vi "ZM-receiver.vi"() -> ()   [LabVIEW 2020]
doc: "UDP receiver of the tree's data: a plain top-level VI outside the actor tree, started and stopped at any time. It listens on port (default 61557), charts temperature_c and duty_percent of each test package, and shows the last line, the packet count and the measured interval; other package types are skipped. Stop or an error ends it and releases the port."
uses:
  protocol/ZM-CP-UDP-udp_transport/ZM-CP-UDP-receiver/ZM-CP-UDP-receiver.lvclass
  common/ZM-PC-packages/ZM-PC-package/ZM-PC-HEADER.ctl
  common/ZM-PC-packages/ZM-PC-package/ZM-PC-package.lvclass
  common/ZM-PC-packages/ZM-PC-TP-test_package/ZM-PC-TP-DATA.ctl
  common/ZM-PC-packages/ZM-PC-TP-test_package/ZM-PC-TP-test_package.lvclass
panel:
  out "error out":errorcluster
  in  "Stop":bool
  out "packets":u32
  out "last line":string
  out "interval measured (ms)":u32
  out "chart":cluster{"temperature_c":dbl, "duty_percent":dbl}(graph)
  in  "port":u16=61557
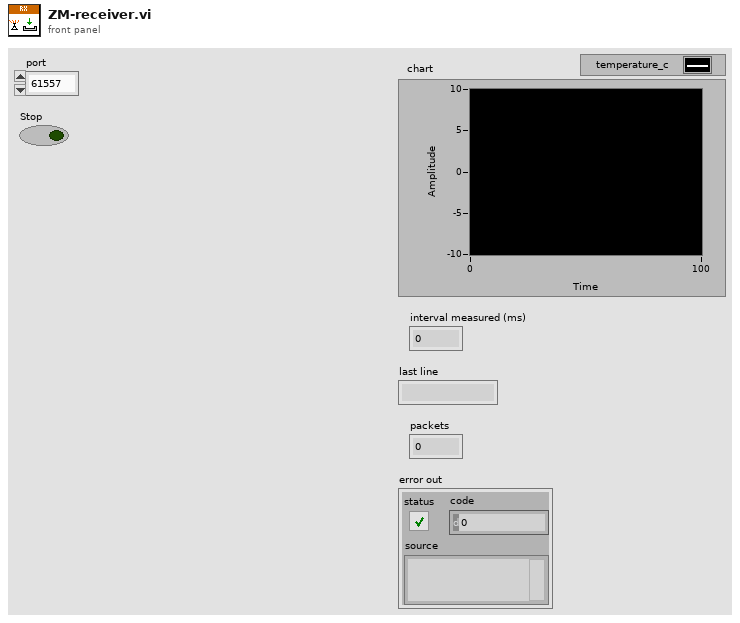
[diagram p1: front panel]
types:
  T1 = typedef "ZM-PC-packages.lvlib/ZM-PC-TP-test_package.lvclass/ZM-PC-TP-DATA.ctl" = cluster{"temperature_c":dbl, "sample_index":i32, "duty_percent":u8, "sensor_ok":bool, "status":string}
  T2 = typedef "ZM-PC-packages.lvlib/ZM-PC-package.lvclass/ZM-PC-HEADER.ctl" = cluster{"timestamp":string, "type":string, "destination":string}
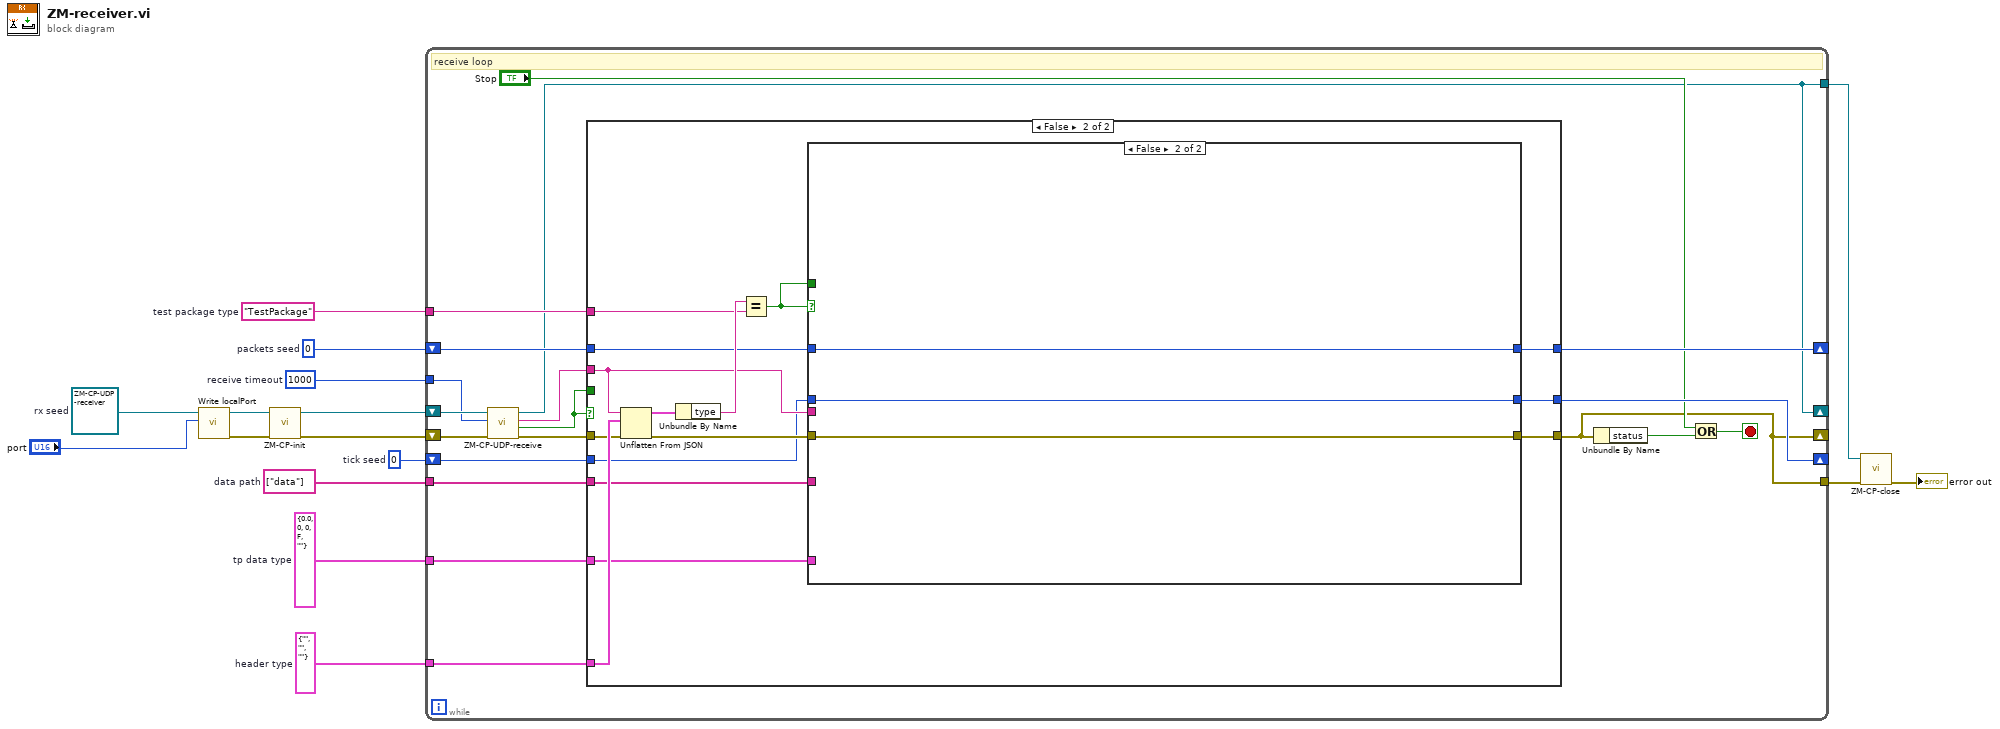
[diagram p0: block diagram]
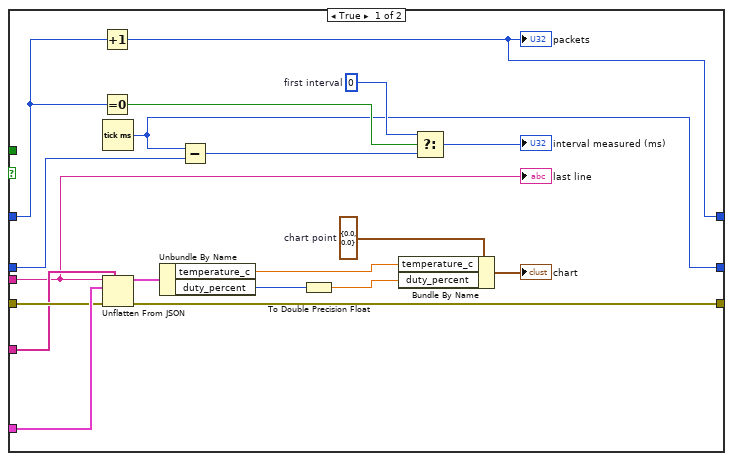
[diagram p3: hidden frame]
diagram:
  w5 = u32 0  # tick seed
  w4 = u32 0  # packets seed
  w8 = "TestPackage"  # test package type
  w9 = 1000  # receive timeout
  w10 = string[] ["data"]  # data path
  w11 = T1 {"temperature_c"=0.0, "sample_index"=0, "duty_percent"=0, "sensor_ok"=FALSE, "status"=""}  # tp data type
  w12 = T2 {"timestamp"="", "type"="", "destination"=""}  # header type
  w16 = refnum<class "ZM-CP-UDP-receiver.lvclass"> refnum  # rx seed
  n1 = call "Write localPort.vi"("localPort"="port", "ZM-CP-UDP-receiver in"=w16) -> ("error out"=w13:errorcluster, "ZM-CP-UDP-receiver out"=w14:refnum<class "ZM-CP-UDP-receiver.lvclass">)  [unwired: 8 in]
  n2 = call-dynamic "ZM-CP-init.vi"("error in (no error)"=w13, "ZM-CP-UDP-receiver in"=w14) -> ("error out"=w6:errorcluster, "ZM-CP-UDP-receiver out"=w7:refnum<class "ZM-CP-UDP-receiver.lvclass">)  [unwired: 8 in]
  n3 = while {
    tunnel: w12 -> [w30]
    tunnel: w11 -> [w29]
    tunnel: w10 -> [w28]
    tunnel: w9 -> [w34]
    tunnel: w8 -> [w27]
    shift-right: [w18] -> _
    shift-left: w7 -> [w35]
    shift-right: [w17] -> _
    shift-left: w6 -> [w33]
    shift-right: [w24] -> _
    shift-left: w5 -> [w26]
    shift-right: [w23] -> _
    shift-left: w4 -> [w25]
    tunnel: [w18] -> w3
    tunnel: [w17] -> w2
    stop <- w19 stop-if-true
    # "receive loop"
    n4 = call "ZM-CP-UDP-receive.vi"("error in (no error)"=w33, "timeout_ms"=w34, "ZM-CP-UDP-receiver in"=w35) -> ("error out"=w32:errorcluster, "timed_out"=w22:bool, "json"=w31:string, "ZM-CP-UDP-receiver out"=w18:refnum<class "ZM-CP-UDP-receiver.lvclass">)  [unwired: 5 in]
    n5 = case shown="False" w22 {
      tunnel: w22 -> [_ _]
      tunnel: w32 -> [w38 w52]
      tunnel: w31 -> [_ w47]
      tunnel: w30 -> [_ w53]
      tunnel: w29 -> [_ w46]
      tunnel: w28 -> [_ w45]
      tunnel: w27 -> [_ w49]
      tunnel: w26 -> [w37 w44]
      tunnel: w25 -> [w36 w43]
      tunnel: [w38 w41] -> w17
      tunnel: [w37 w40] -> w24
      tunnel: [w36 w39] -> w23
      frame True {
      }
      frame False {
        n6 = Unflatten From JSON(JSON string=w47, type and defaults=w53, error in (no error)=w52) -> (value=w51:T2, error out=w48:errorcluster)  [unwired: 4 in]
        n7 = Unbundle By Name(w51) -> ("type"=w50:string)
        n8 = Equal?(x=w50, y=w49) -> (x = y?=w42:bool)
        n9 = case shown="False" w42 {
          tunnel: w42 -> [_ _]
          tunnel: w48 -> [w71 w75]
          tunnel: w47 -> [w58 _]
          tunnel: w46 -> [w72 _]
          tunnel: w45 -> [w70 _]
          tunnel: w44 -> [w63 w74]
          tunnel: w43 -> [w57 w73]
          tunnel: [w56 w75] -> w41
          tunnel: [w55 w74] -> w40
          tunnel: [w54 w73] -> w39
          frame True {
            w62 = u32 0  # first interval
            w65 = cluster{"temperature_c":dbl, "duty_percent":dbl} {"temperature_c"=0.0, "duty_percent"=0.0}  # chart point
            n10 = Increment(x=w57) -> (x+1=w54:u32)
            "packets" <- w54
            n11 = Equal To 0?(x=w57) -> (x = 0?=w61:bool)
            n12 = Tick Count (ms)() -> (millisecond timer value=w55:u32)
            n13 = Unflatten From JSON(path=w70, JSON string=w58, type and defaults=w72, error in (no error)=w71) -> (value=w69:T1, error out=w56:errorcluster)  [unwired: 3 in]
            n14 = Unbundle By Name(w69) -> ("temperature_c"=w67:dbl, "duty_percent"=w68:u8)
            n15 = Subtract(x=w55, y=w63) -> (x-y=w60:u32)
            n16 = To Double Precision Float(number=w68) -> (double precision float=w66:dbl)
            n17 = Bundle By Name(cluster=w65, "temperature_c"=w67, "duty_percent"=w66) -> (→"chart":cluster{"temperature_c":dbl, "duty_percent":dbl})
            n18 = Select(t=w62, s=w61, f=w60) -> (s? t:f=→"interval measured (ms)":u32)
            "last line" <- w58
          }
          frame False {
          }
        }
      }
    }
    n19 = Unbundle By Name(w17) -> ("status"=w20:bool)
    n20 = Or(x="Stop", y=w20) -> (x .or. y?=w19:bool)
  }
  n21 = call-dynamic "ZM-CP-close.vi"("error in (no error)"=w2, "ZM-CP-UDP-receiver in"=w3) -> ("error out"=→"error out":errorcluster)  [unwired: 8 in, 1 out]
